vi ".vi"(0 "error in (no escape)":errorcluster) -> ()   [LabVIEW 2020]
doc: "\"The rabbit-hole went straight on like a tunnel for some way, and then dipped suddenly down, so suddenly that Alice had not a moment to think about stopping herself before she found herself falling down a very deep well.\""
panel:
  # "\"But I don't want to go among mad people,\" Alice remarked.\n\n\"Oh, you can’t help that,\" said the Cat: \"we're all mad here. I'm mad. You're mad.\"\n\n\"How do you know I'm mad?\" said Alice.\n\n\"You must be,\" said the Cat, \"or you wouldn't have come here.\"\n\n                                                              - Alice's Adventures in LabVIEWland"
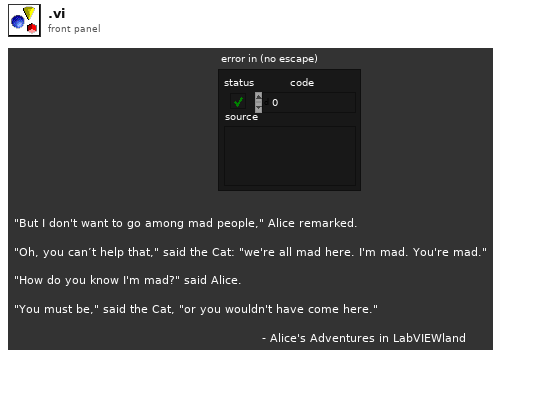
[diagram p1: front panel]
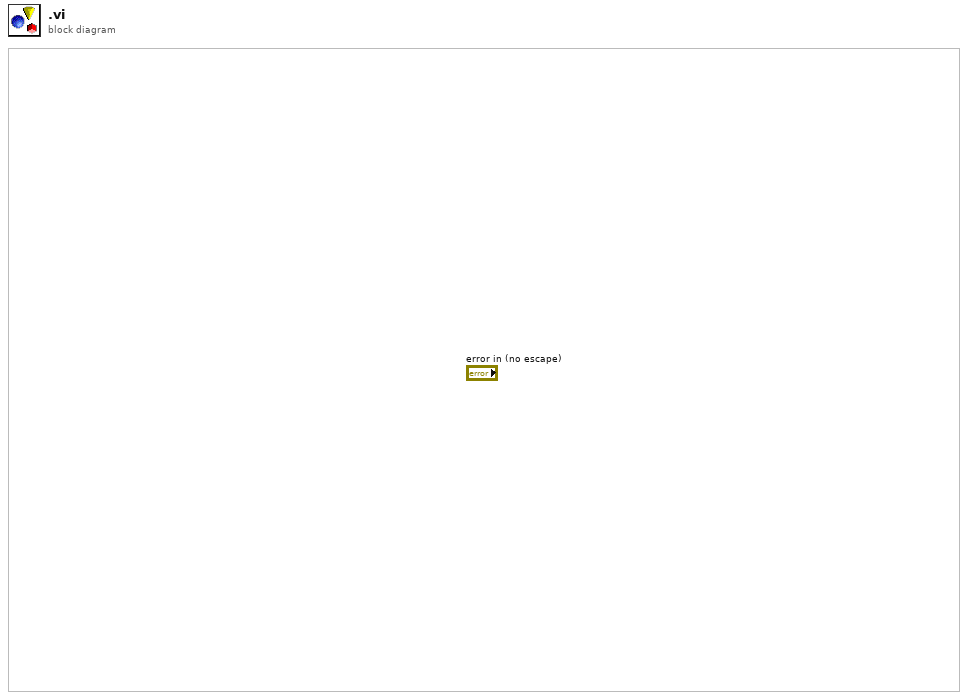
[diagram p0: block diagram]
diagram:
